vi "Throw Index Out Of Bounds Error.vi"(8 "Error In":errorcluster) -> (0 "Error Out":errorcluster caption="Error Out\nThis indicator is larger than usual in order to enable the viewing of the whole error message.")   [LabVIEW 2026, in "RSysUtils Array.lvlib"]
doc: "This VI throws, raises or outputs an error with:\nError Code = 5001 (distinctive error code)\nError Message = \"Index was outside the bounds of the array.\"\n\nIf the \"Error In\" input already carries an error, this VI forwards that error to \"Error Out\" unaltered. It does not overwrite input errors."
uses:
  RSysUtils Array.lvlib
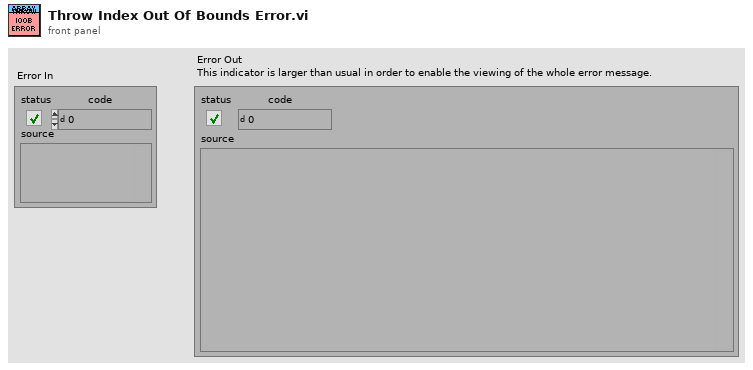
[diagram p1: front panel]
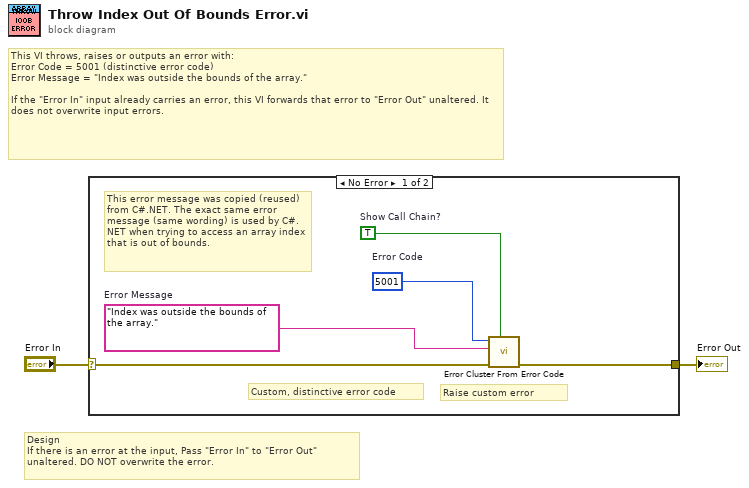
[diagram p0: block diagram]
diagram:
  # "This VI throws, raises or outputs an error with:\nError Code = 5001 (distinctive error code)\nError Message = \"Index was outside the bounds of the array.\"\n\nIf the \"Error In\" input already carries an error, this VI forwards that error to \"Error Out\" unaltered. It does not overwrite input errors."
  # "Design\nIf there is an error at the input, Pass \"Error In\" to \"Error Out\" unaltered. DO NOT overwrite the error."
  n1 = case shown="No Error" "Error In" {
    selector: "Error In" -> [w6 w8]
    tunnel: [w7 w8] -> w2
    frame No Error {
      w3 = TRUE  # Show Call Chain?
      w4 = "Index was outside the bounds of the array."  # Error Message
      w5 = 5001  # Error Code
      # "Custom, distinctive error code"
      # "This error message was copied (reused) from C#.NET. The exact same error message (same wording) is used by C#.NET when trying to access an array index that is out of bounds."
      # "Raise custom error"
      n2 = call <vilib>:"Error Cluster From Error Code.vi"("show call chain? (False)"=w3, "error in (no error)"=w6, "error message (\"\")"=w4, "error code (0)"=w5) -> ("error out"=w7:errorcluster)  [unwired: 5 in]
    }
    frame Error {
      # "There is an input error. Do nothing. Pass error along. Do not overwrite."
    }
  }
  "Error Out" <- w2
